vi "2.gauss_fit.vi"() -> ()   [LabVIEW 2017]
panel:
  out "size(s)":i32
  out "appended array":dbl[](array[numeric])
  out "x-y":dbl
  in  "end":dbl
  in  "start":dbl
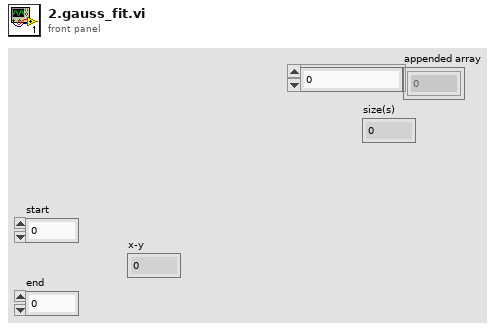
[diagram p1: front panel]
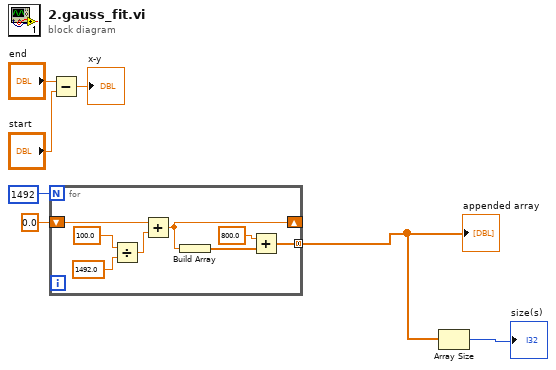
[diagram p0: block diagram]
diagram:
  n1 = for {
    N: 1492 -> [_]
    shift-right: [w14] -> _
    shift-left: 0.0 -> [w15]
    tunnel: [w11] -> w2 mode=concatenating
    n2 = Divide(x=100.0 ("x/y"), y=1492.0) -> (x/y=w8:dbl)
    n3 = Add(x=w15, y=w8) -> (x+y=w14:dbl)
    n4 = Build Array(w14) -> (w12:dbl[])
    n5 = Add(x=800.0 ("x+y"), y=w12) -> (x+y=w11:dbl[])
  }
  "appended array" <- w2
  n6 = Subtract(x="end", y="start") -> (x-y=→"x-y":dbl)
  n7 = Array Size(array=w2) -> (size(s)=→"size(s)":i32)
